vi "thermal_1.vi"() -> ()   [LabVIEW 2025]
panel:
  out "Image":T1(plugin-control)
  in  "Stop Preview":bool
  in  "STOP ACQUISITION":bool
  in  "Focus":dbl(slide) scale=0.0..100.0
  out "Thermal Frame Out":string
  in  "Output Folder":path
  in  "thermal capture interval (s)":dbl
  in  "Flag Button":bool
  in  "Stop & Save":bool
  in  "Record":bool
  # "(1) Run VI"
  # "(2) After thermal camera calibration message (in terminal), press START"
  # "(3) Stop & Save"
  # "THERMAL CONTROLS"
  # "(Enter \"28\")"
  # "Thermal Record"
  # "OPTICAL CONTROLS"
  # "(must be an empty folder)"
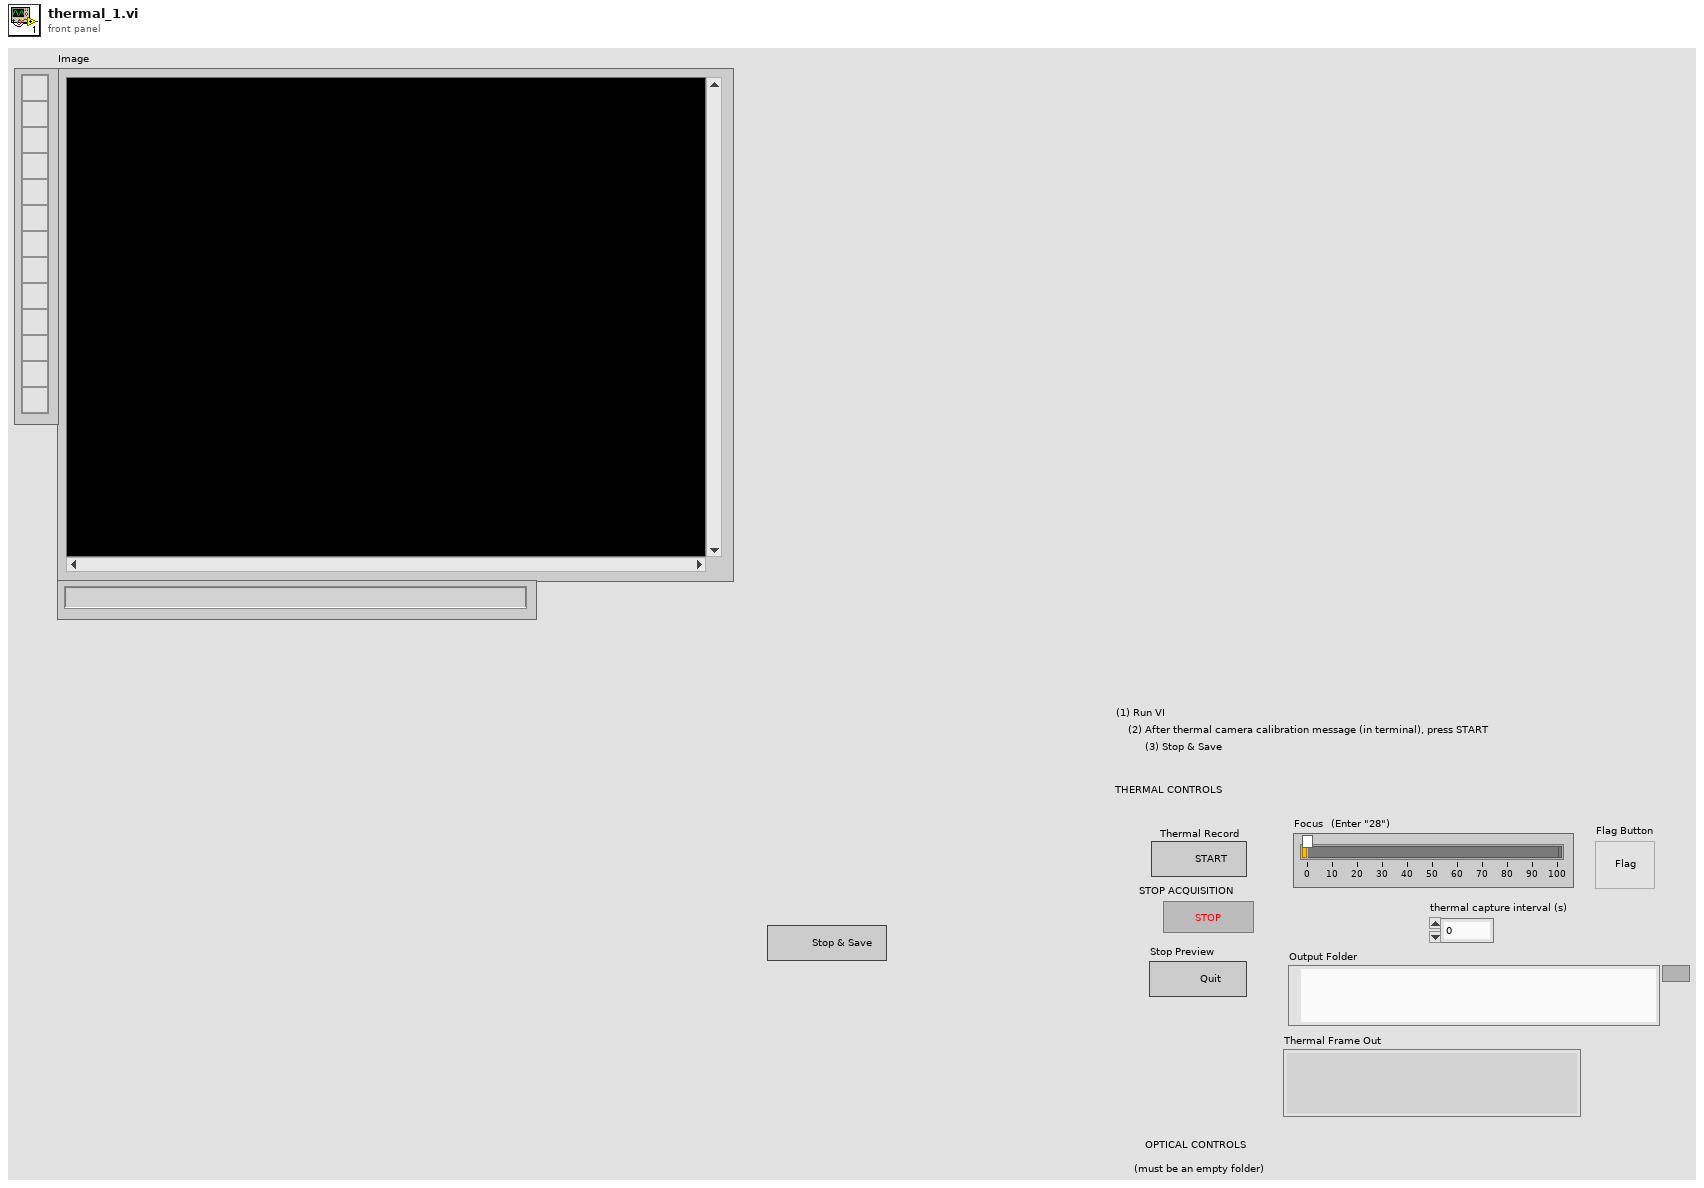
[diagram p1: front panel]
types:
  T1 = typedef "IMAQ Image.ctl" = refnum<image>
  T2 = enum16{"open", "replace", "create", "open or create", "replace or create", "replace or create with confirmation"}
  T3 = enum16{"big-endian, network order", "native, host order", "little-endian"}
  T4 = typedef "Image Type" = u32
  T5 = enum16{"Standard", "Buffered", "CRLF", "Immediate"}
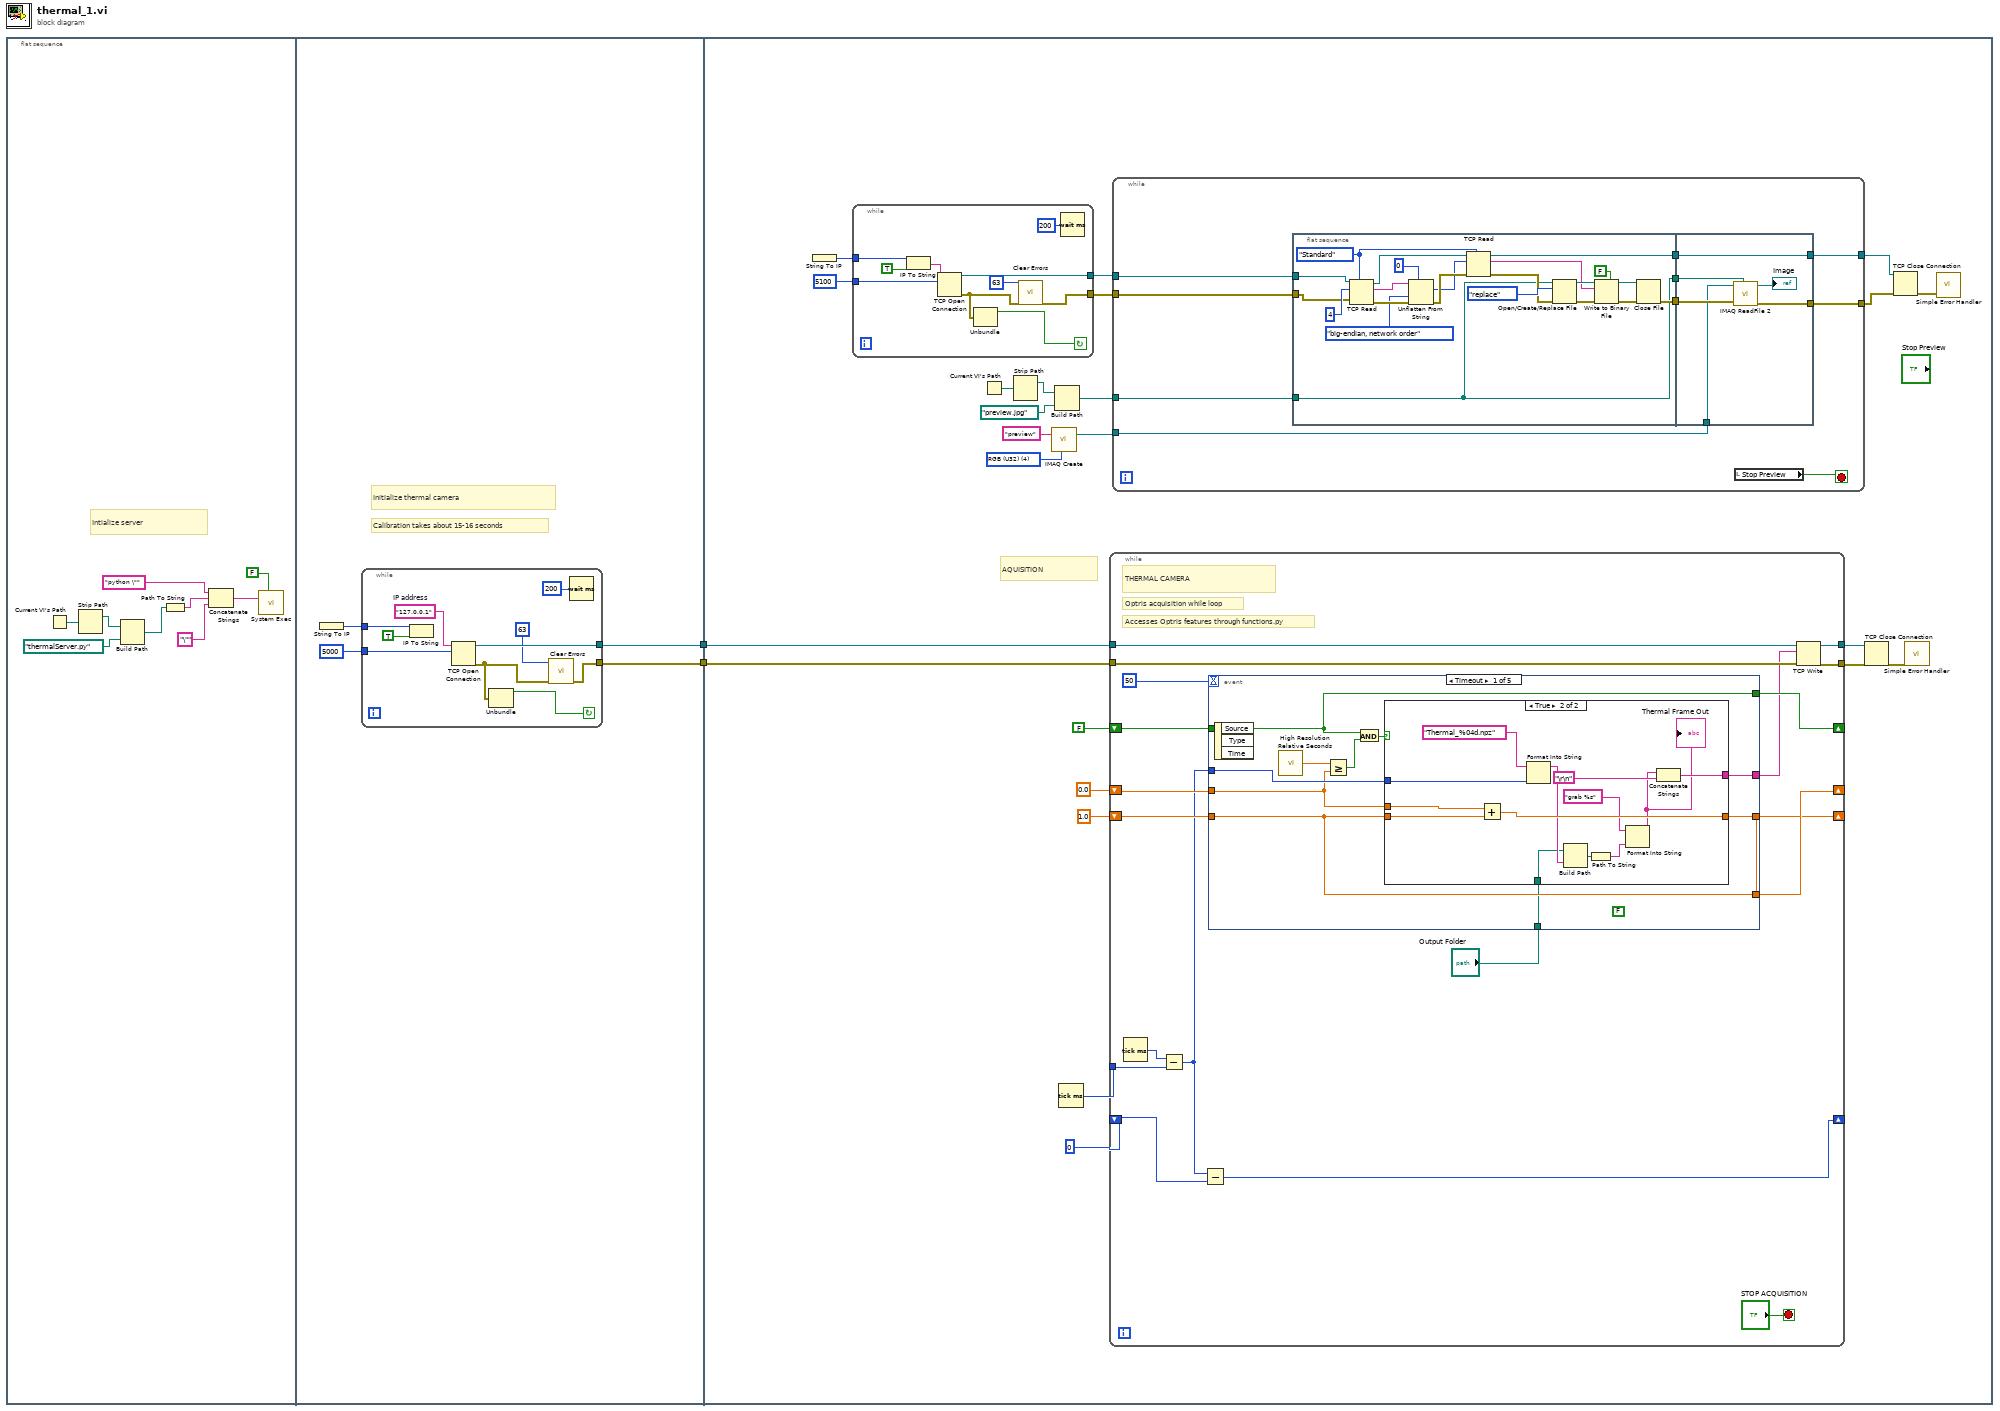
[diagram p0: block diagram]
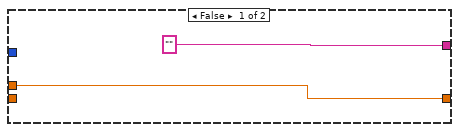
[diagram p2: hidden frame]
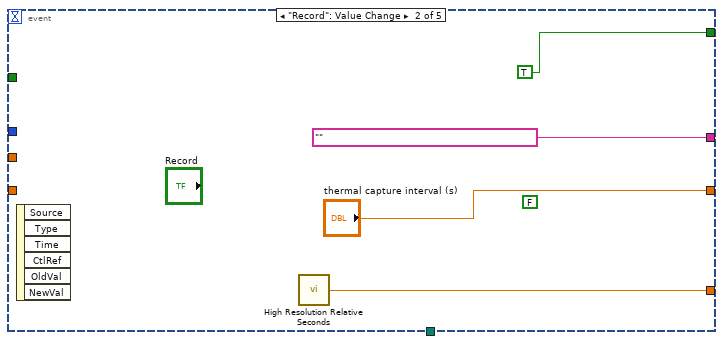
[diagram p3: hidden frame]
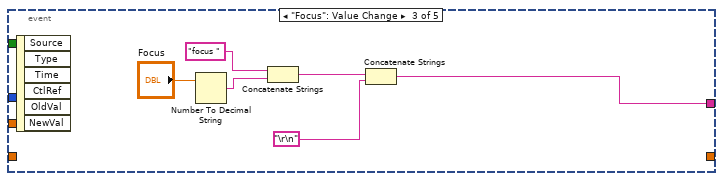
[diagram p4: hidden frame]
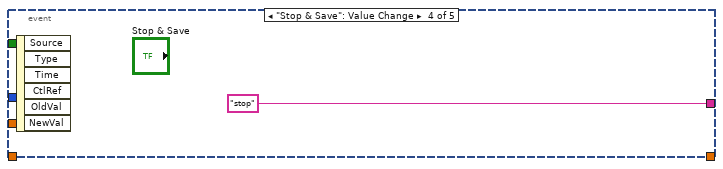
[diagram p5: hidden frame]
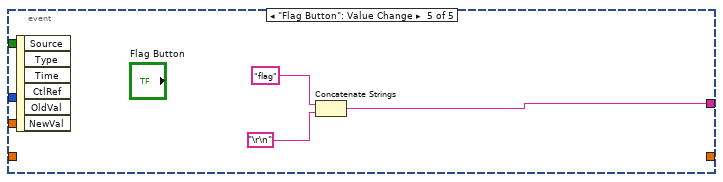
[diagram p6: hidden frame]
diagram:
  n1 = flat-sequence {
    tunnel: [w13] -> w2
    tunnel: [w12] -> w1
    tunnel: w1 -> [w46]
    tunnel: w2 -> [w45]
    frame #0 {
      # "Intialize server"
      n2 = Current VI's Path() -> (path=w6:path)
      n3 = Strip Path(path=w6) -> (stripped path=w7:path)  [unwired: 1 out]
      n4 = Build Path(base path=w7, name or relative path=path "thermalServer.py") -> (appended path=w4:path)
      n5 = Path To String(path=w4) -> (string=w10:string)
      n6 = Concatenate Strings("python \"" ("string"), w10, "\"" ("string")) -> (w9:string)
      n7 = call <vilib>:"System Exec.vi"("wait until completion? (T)"=FALSE, "command line"=w9) -> ()  [unwired: 6 in, 4 out]
    }
    frame #1 {
      # "Initialize thermal camera"
      # "Calibration takes about 15-16 seconds"
      n8 = String To IP() -> (0:w15:u32)  [unwired: 1 in]
      n9 = while {
        tunnel: [w20] -> w13
        tunnel: [w25] -> w12
        tunnel: w15 -> [w24]
        tunnel: u16 5000 ("remote port or service name") -> [w22]
        stop <- w17 continue-if-true
        w16 = "127.0.0.1"  # IP address
        n10 = IP To String(1:TRUE ("dot notation? (F)"), 2:w24) -> ()  [unwired: 1 out]
        n11 = TCP Open Connection(address=w16, remote port or service name=w22) -> (connection ID=w25:refnum<k5>, error out=w21:errorcluster)  [unwired: 3 in]
        n12 = Unbundle(w21) -> ("status"=w17:bool)  [unwired: 2 out]
        n13 = call <vilib>:"Clear Errors.vi"("error in (no error)"=w21, "specific error code to clear (0: all)"=63) -> ("error out"=w20:errorcluster)  [unwired: 4 in, 1 out]
        n14 = Wait (ms)(milliseconds to wait=u32 200) -> ()  [unwired: 1 out]
      }
    }
    frame #2 {
      w30 = T4 4 items=["Grayscale (U8)", "Grayscale (I16)", "Grayscale (SGL)", "Complex (CSG)", "RGB (U32)", "HSL (U32)", "RGB (U64)", "Grayscale (U16)"] ("Image Type")
      # "AQUISITION"
      n15 = String To IP() -> (0:w29:u32)  [unwired: 1 in]
      n16 = while {
        tunnel: w29 -> [w59]
        tunnel: [w53] -> w28
        tunnel: [w57] -> w27
        tunnel: u16 5100 ("remote port or service name") -> [w55]
        stop <- w50 continue-if-true
        n17 = IP To String(1:TRUE ("dot notation? (F)"), 2:w59) -> (0:w58:string)
        n18 = TCP Open Connection(address=w58, remote port or service name=w55) -> (connection ID=w57:refnum<k5>, error out=w54:errorcluster)  [unwired: 3 in]
        n19 = Unbundle(w54) -> ("status"=w50:bool)  [unwired: 2 out]
        n20 = call <vilib>:"Clear Errors.vi"("error in (no error)"=w54, "specific error code to clear (0: all)"=63) -> ("error out"=w53:errorcluster)  [unwired: 4 in, 1 out]
        n21 = Wait (ms)(milliseconds to wait=u32 200) -> ()  [unwired: 1 out]
      }
      n22 = Current VI's Path() -> (path=w38:path)
      n23 = Strip Path(path=w38) -> (stripped path=w39:path)  [unwired: 1 out]
      n24 = call "IMAQ Create"("Image Name"="preview", "Image Type"=w30) -> ("New Image"=w34:T1)  [unwired: 3 in, 1 out]
      n25 = Build Path(base path=w39, name or relative path=path "preview.jpg") -> (appended path=w37:path)
      n26 = Tick Count (ms)() -> (millisecond timer value=w41:u32)
      n27 = while {
        tunnel: [w116] -> w47
        tunnel: [w115] -> w48
        tunnel: w46 -> [w114]
        tunnel: w45 -> [w113]
        shift-right: [w112] -> _
        shift-left: 0.0 -> [w108]
        shift-right: [w109] -> _
        shift-left: 1.0 -> [w106]
        shift-right: [w110] -> _
        shift-left: FALSE -> [w107]
        tunnel: w41 -> [w102]
        shift-right: [w98] -> _
        shift-left: u32 0 -> [w100]
        stop <- "STOP ACQUISITION" stop-if-true
        # "THERMAL CAMERA"
        # "Optris acquisition while loop"
        # "Accesses Optris features through functions.py"
        n28 = Tick Count (ms)() -> (millisecond timer value=w103:u32)
        n29 = Subtract(x=w103, y=w102) -> (x-y=w101:u32)
        n30 = Subtract(x=w101, y=w100) -> (x-y=w98:u32)
        n31 = event shown="[0] Timeout" {
          selector: _ -> [_ _ _ _ _]
          dyn-events: _ -> [_ _ _ _ _]
          timeout: 50 -> [_ _ _ _ _]
          tunnel: [w122 "" w146 "stop" w155] -> w105
          tunnel: w101 -> [w123 _ _ _ _]
          tunnel: [w120 w145 _ _ _] -> w112
          tunnel: [w118 TRUE _ _ _] -> w110
          tunnel: [w119 "thermal capture interval (s)" _ _ _] -> w109
          tunnel: w108 -> [w121 _ _ _ _]
          tunnel: w107 -> [w118 _ _ _ _]
          tunnel: w106 -> [w119 _ _ _ _]
          tunnel: "Output Folder" -> [w117 _ _ _ _]
          event Timeout {
            (unwired) FALSE
            n32 = event-data() -> ()  [unwired: 1 in, 3 out]
            n33 = call <vilib>:"High Resolution Relative Seconds.vi"() -> ("relative seconds"=w126:dbl)
            n34 = Greater Or Equal?(x=w126, y=w121) -> (x >= y?=w125:bool)
            n35 = And(x=w118, y=w125) -> (x .and. y?=w124:bool)
            n36 = case shown="True" w124 {
              tunnel: w123 -> [_ w139]
              tunnel: ["" w140] -> w122
              tunnel: w121 -> [w127 w138]
              tunnel: w119 -> [_ w137]
              tunnel: [w127 w136] -> w120
              tunnel: w117 -> [_ w129]
              frame False {
              }
              frame True {
                n37 = Add(x=w138, y=w137) -> (x+y=w136:dbl)
                n38 = Format Into String(format string="Thermal_%04d.npz", w139) -> (resulting string=w132:string)  [unwired: 2 in, 1 out]
                n39 = Build Path(base path=w129, name or relative path=w132) -> (appended path=w134:path)
                n40 = Path To String(path=w134) -> (string=w131:string)
                n41 = Format Into String(format string="grab %s", w131) -> (resulting string=w130:string)  [unwired: 2 in, 1 out]
                "Thermal Frame Out" <- w130
                n42 = Concatenate Strings(w130, "\r\n") -> (w140:string)
              }
            }
          }
          event "Record": Value Change {
            (unwired) FALSE
            n43 = event-data() -> ()  [unwired: 1 in, 6 out]
            n44 = call <vilib>:"High Resolution Relative Seconds.vi"() -> ("relative seconds"=w145:dbl)
          }
          event "Focus": Value Change {
            n45 = event-data() -> ()  [unwired: 1 in, 6 out]
            n46 = Number To Decimal String(number="Focus") -> (decimal integer string=w151:string)  [unwired: 1 in]
            n47 = Concatenate Strings("focus ", w151) -> (w148:string)
            n48 = Concatenate Strings(w148, "\r\n") -> (w146:string)
          }
          event "Stop & Save": Value Change {
            n49 = event-data() -> ()  [unwired: 1 in, 6 out]
          }
          event "Flag Button": Value Change {
            n50 = event-data() -> ()  [unwired: 1 in, 6 out]
            n51 = Concatenate Strings("flag", "\r\n") -> (w155:string)
          }
        }
        n52 = TCP Write(connection ID=w114, data in=w105, error in (no error)=w113) -> (connection ID out=w115:refnum<k5>, error out=w116:errorcluster)  [unwired: 1 in, 1 out]
      }
      n53 = while {
        tunnel: w34 -> [w64]
        tunnel: [w65] -> w35
        tunnel: [w69] -> w36
        tunnel: w37 -> [w67]
        tunnel: w28 -> [w62]
        tunnel: w27 -> [w61]
        stop <- w60 stop-if-true
        n54 = flat-sequence {
          tunnel: w67 -> [w73]
          tunnel: [w75] -> w68
          tunnel: [w74] -> w66
          tunnel: [w73] -> w63
          tunnel: w62 -> [w71]
          tunnel: w61 -> [w70]
          tunnel: [w97] -> w69
          tunnel: w68 -> [w97]
          tunnel: w66 -> [w96]
          tunnel: [w95] -> w65
          tunnel: w64 -> [w94]
          tunnel: w63 -> [w93]
          frame #0 {
            w84 = T5."Standard" ("mode (standard)")
            n55 = TCP Read(connection ID=w70, bytes to read=4, error in (no error)=w71, 7:w84) -> (connection ID out=w87:refnum<k5>, data out=w72:string, error out=w90:errorcluster)  [unwired: 1 in]
            n56 = Unflatten From String(type=0, binary string=w72, byte order (0:big-endian, network order)=T3."big-endian, network order", error in (no error)=w90) -> (value=w85:i32, error out=w86:errorcluster)  [unwired: 1 in, 1 out]
            n57 = TCP Read(connection ID=w87, bytes to read=w85, error in (no error)=w86, 7:w84) -> (connection ID out=w75:refnum<k5>, data out=w80:string, error out=w82:errorcluster)  [unwired: 1 in]
            n58 = Open/Create/Replace File(file path (use dialog)=w73, error in=w82, operation (0:open)=T2."replace") -> (refnum out=w81:refnum<file>, error out=w78:errorcluster)  [unwired: 3 in, 1 out]
            n59 = Write to Binary File(file (use dialog)=w81, data=w80, error in=w78, 5:FALSE ("prepend array or string size? (T)")) -> (refnum out=w76:refnum<file>, error out=w77:errorcluster)  [unwired: 2 in, 1 out]
            n60 = Close File(refnum=w76, error in=w77) -> (error out=w74:errorcluster)  [unwired: 1 out]
          }
          frame #1 {
            n61 = call "IMAQ ReadFile 2"("File Path"=w93, "error in (no error)"=w96, "Image"=w94) -> ("error out"=w95:errorcluster, "Image Out"=→"Image":T1)  [unwired: 4 in, 3 out]
          }
        }
        n62 = local read "Stop Preview"() -> (w60:bool)
      }
      n63 = TCP Close Connection(connection ID=w48, error in (no error)=w47) -> (error out=w49:errorcluster)  [unwired: 1 in, 1 out]
      n64 = TCP Close Connection(connection ID=w36, error in (no error)=w35) -> (error out=w33:errorcluster)  [unwired: 1 in, 1 out]
      n65 = call <vilib>:"Simple Error Handler.vi"("error in (no error)"=w49) -> ()  [unwired: 4 in, 5 out]
      n66 = call <vilib>:"Simple Error Handler.vi"("error in (no error)"=w33) -> ()  [unwired: 4 in, 5 out]
    }
  }
